vi "add.vi"(9 "x":dbl, 11 "y":dbl) -> (2 "x+y":dbl)   [LabVIEW 2017]
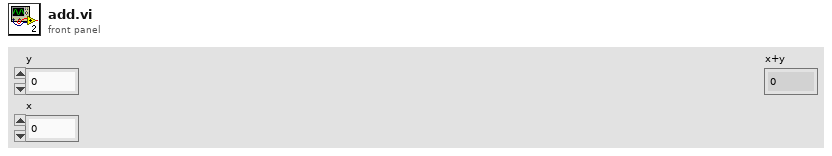
[diagram p1: front panel]
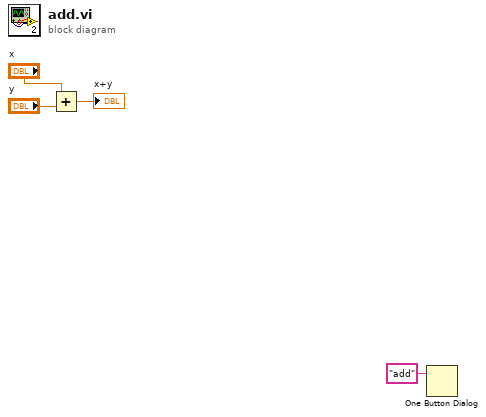
[diagram p0: block diagram]
diagram:
  n1 = Add(x="x", y="y") -> (x+y=→"x+y":dbl)
  n2 = One Button Dialog(message="add") -> ()  [unwired: 1 in, 1 out]
